vi "Write Projects.vi"(8 "error in (no error)":errorcluster, 10 "Project List":T1, 11 "Project Store in":refnum<class "Project Store.lvclass">) -> (0 "error out":errorcluster, 3 "Project Store out":refnum<class "Project Store.lvclass">)   [LabVIEW 2024, in "Project Store.lvclass"]
doc: "Writes one field of this class's private data. Generated by lvai_create_accessors from the class private data control."
uses:
  Project Store.lvclass
  Project Store.lvclass/Project Store.ctl
  Rows/Project.ctl
  Rows/Project List.ctl
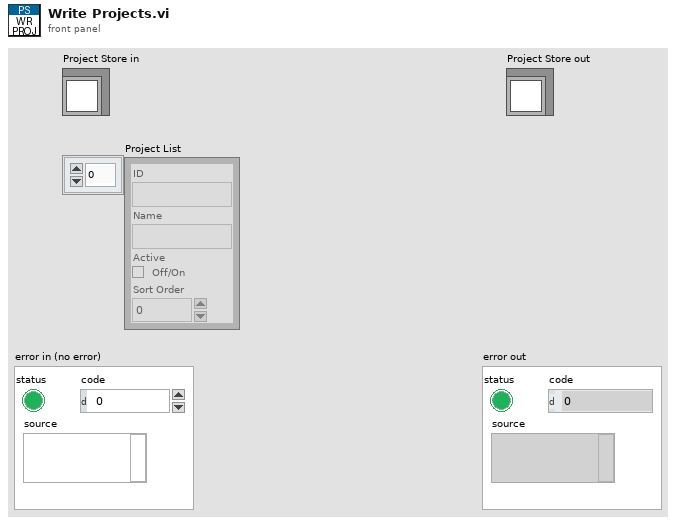
[diagram p1: front panel]
types:
  T1 = typedef "Project List.ctl" = T2[]
  T2 = typedef "Project.ctl" = cluster{"ID":string, "Name":string, "Active":bool, "Sort Order":i32}
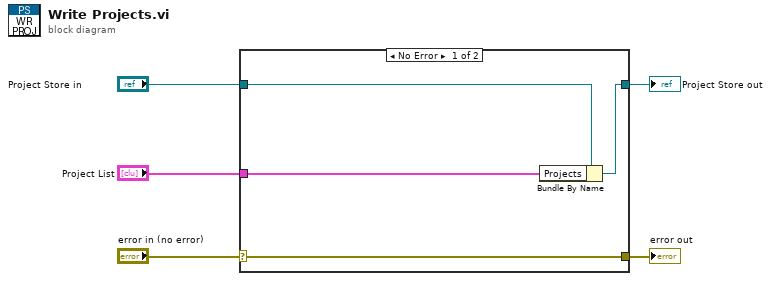
[diagram p0: block diagram]
diagram:
  n1 = case shown="No Error" "error in (no error)" {
    selector: "error in (no error)" -> [w9 w10]
    tunnel: [w9 w10] -> w4
    tunnel: [w7 w11] -> w2
    tunnel: "Project Store in" -> [w8 w11]
    tunnel: "Project List" -> [w6 _]
    frame No Error {
      n2 = Bundle By Name(cluster=w8, "Projects"=w6) -> (w7:refnum<class "Project Store.lvclass">)
    }
    frame Error {
    }
  }
  "error out" <- w4
  "Project Store out" <- w2
